vi "Capture_Abort.vi"(8 "error in (no error)":errorcluster={"status"=FALSE, "code"=0, "source"="\"\""}, 10 "reason":string, 11 "Session ID":string) -> (0 "error out":errorcluster={"status"=FALSE, "code"=0, "source"="\"\""}, 2 "status ok":bool, 3 "Partial result":string)   [LabVIEW 2026]
doc: "INTENT: Terminate capture on fault/cancel. LOGIC: Stop session, flag incomplete and publish partial data policy."
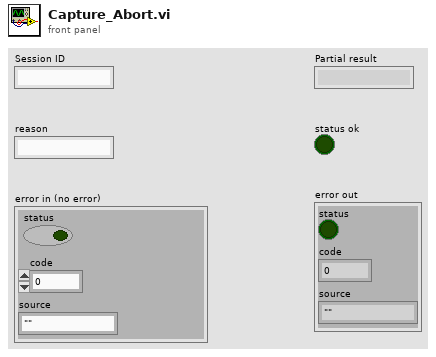
[diagram p1: front panel]
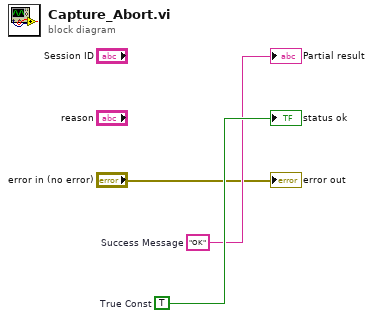
[diagram p0: block diagram]
diagram:
  w3 = TRUE  # True Const
  w2 = "OK"  # Success Message
  "Partial result" <- w2
  "status ok" <- w3
  "error out" <- "error in (no error)"
